vi "Tachomodus (SubVI).vi"(0 "Lambda":refnum<vi>, 4 "EGT":refnum<vi>, 5 "AFR EGT":refnum<vi>, 6 "AFR":refnum<vi>, 7 "cvt":bool, 8 "Leistung":refnum<vi>, 9 "Stopp":refnum<vi>, 10 "Hinterrad":refnum<vi>, 11 "Welle":refnum<vi>) -> ()   [LabVIEW 2014]
panel:
  in  "Text Rolle":string="Rolle"
  in  "Text Zündung":string="Zündung"
  out "Welle [1/min]\n[1/min]":cluster{dbl, dbl}(knob) caption="Welle\n[1/min]" scale=0.0..14000.0
  out "Hinterrad (Tacho)\n[km/h]":dbl(knob) caption="Hinterrad\n[km/h]" scale=0.0..200.0
  out "EGT\n[°C]":dbl(knob) scale=0.0..800.0 scale format="%#.6g"
  out "AFR":dbl(knob) scale=10.0..20.0
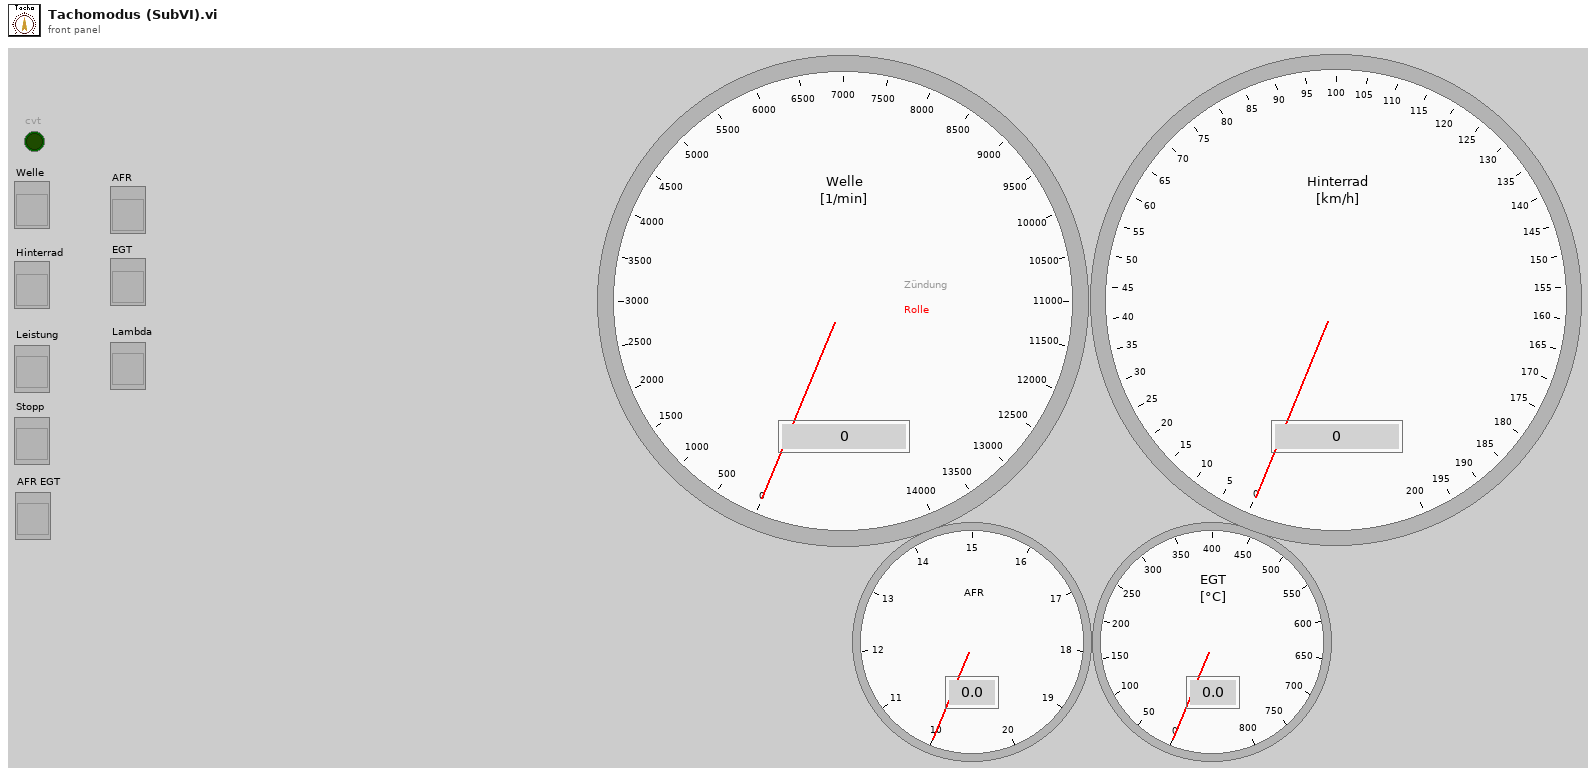
[diagram p1: front panel]
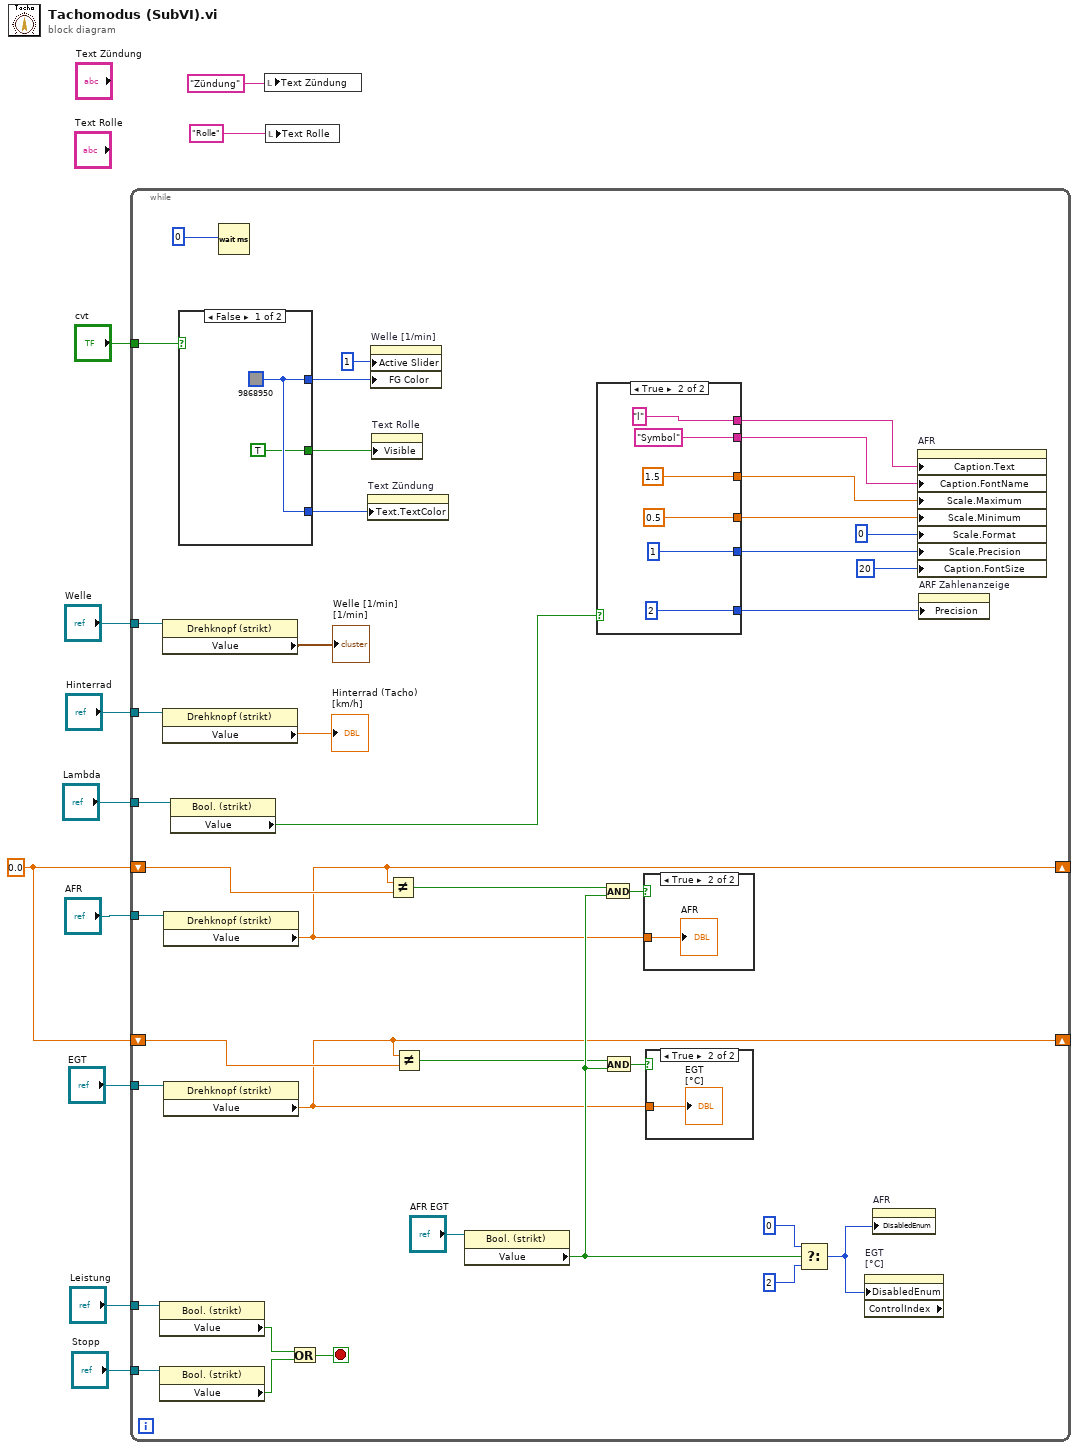
[diagram p0: block diagram]
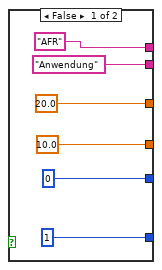
[diagram p2: hidden frame]
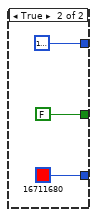
[diagram p5: hidden frame]
diagram:
  w2 = 0.0
  n1 = while {
    tunnel: "Welle" -> [w51]
    tunnel: "Hinterrad" -> [w50]
    tunnel: "Leistung" -> [w49]
    tunnel: "Stopp" -> [w47]
    tunnel: "cvt" -> [w44]
    tunnel: "AFR" -> [w36]
    tunnel: "EGT" -> [w35]
    shift-right: [w13] -> _
    shift-left: w2 -> [w30]
    shift-right: [w23] -> _
    shift-left: w2 -> [w24]
    tunnel: "Lambda" -> [w22]
    stop <- w46 stop-if-true
    n2 = property class="Bool. (strikt)"(reference=w49) -> ("Value"=w48:bool)  [unwired: 1 in, 2 out]
    n3 = property class="Bool. (strikt)"(reference=w47) -> ("Value"=w45:bool)  [unwired: 1 in, 2 out]
    n4 = property class="Drehknopf (strikt)"(reference=w51) -> ("Value"=→"Welle [1/min]\n[1/min]":cluster{dbl, dbl})  [unwired: 1 in, 2 out]
    n5 = property class="Drehknopf (strikt)"(reference=w50) -> ("Value"=→"Hinterrad (Tacho)\n[km/h]":dbl)  [unwired: 1 in, 2 out]
    n6 = property class="Drehknopf (strikt)"(reference=w36) -> ("Value"=w13:dbl)  [unwired: 1 in, 2 out]
    n7 = property class="Drehknopf (strikt)"(reference=w35) -> ("Value"=w23:dbl)  [unwired: 1 in, 2 out]
    n8 = property class="Bool. (strikt)"(reference=w22) -> ("Value"=w20:bool)  [unwired: 1 in, 2 out]
    n9 = case shown="False" w44 {
      tunnel: [w67 u32 16711680] -> w43
      tunnel: [w67 u32 16777216] -> w41
      tunnel: [TRUE FALSE] -> w40
      frame False {
        w67 = u32 9868950
      }
      frame True {
      }
    }
    n10 = Wait (ms)(milliseconds to wait=0) -> ()  [unwired: 1 out]
    n11 = Or(x=w48, y=w45) -> (x .or. y?=w46:bool)
    n12 = property on="Text Zündung" class="Str"("Text.TextColor"=w43) -> ()  [unwired: 2 in, 2 out]
    n13 = property on="Welle [1/min]" class="Drehknopf (strikt)"("Active Slider"=1, "FG Color"=w41) -> ()  [unwired: 2 in, 2 out]
    n14 = property on="Text Rolle" class="Str"("Visible"=w40) -> ()  [unwired: 2 in, 2 out]
    n15 = Not Equal?(x=w13, y=w30) -> (x != y?=w28:bool)
    n16 = Not Equal?(x=w23, y=w24) -> (x != y?=w25:bool)
    n17 = property class="Bool. (strikt)"(reference="AFR EGT") -> ("Value"=w26:bool)  [unwired: 1 in, 2 out]
    n18 = case shown="True" w20 {
      tunnel: ["AFR" "l"] -> w19
      tunnel: ["Anwendung" "Symbol"] -> w18
      tunnel: [20.0 1.5] -> w17
      tunnel: [10.0 0.5] -> w16
      tunnel: [0 1] -> w15
      tunnel: [1 2] -> w14
      frame False {
      }
      frame True {
      }
    }
    n19 = And(x=w28, y=w26) -> (x .and. y?=w29:bool)
    n20 = And(x=w25, y=w26) -> (x .and. y?=w27:bool)
    n21 = case shown="True" w29 {
      tunnel: w13 -> [_ w65]
      frame False {
      }
      frame True {
        "AFR" <- w65
      }
    }
    n22 = case shown="True" w27 {
      tunnel: w23 -> [_ w64]
      frame False {
      }
      frame True {
        "EGT\n[°C]" <- w64
      }
    }
    n23 = Select(t=0, s=w26, f=2) -> (s? t:f=w33:i32)
    n24 = property on="EGT\n[°C]" class="Drehknopf (strikt)" props=["DisabledEnum", "ControlIndex"]("DisabledEnum"=w33) -> ()  [unwired: 2 in, 3 out]
    n25 = property on="AFR" class="Drehknopf (strikt)"("DisabledEnum"=w33) -> ()  [unwired: 2 in, 2 out]
    n26 = property on="AFR" class="Drehknopf (strikt)"("Caption.Text"=w19, "Caption.FontName"=w18, "Scale.Maximum"=w17, "Scale.Minimum"=w16, "Scale.Format"=0, "Scale.Precision"=w15, "Caption.FontSize"=20) -> ()  [unwired: 2 in, 2 out]
    n27 = property on="ARF Zahlenanzeige" class="DigWert (strikt)"("Precision"=w14) -> ()  [unwired: 2 in, 2 out]
  }
  n28 = local write "Text Zündung"("Zündung") -> ()
  n29 = local write "Text Rolle"("Rolle") -> ()
